vi "_Subsystem_Name Build Trace String.vi"(10 "Current Command":T1, 11 "Initial Trace String":string) -> (3 "Trace String":string)   [LabVIEW 2023]
doc: "This VI is called to construct a trace string from the command arguments."
uses:
  _Subsystem_Name Operations.ctl
  _Subsystem_Name Setpoints.ctl
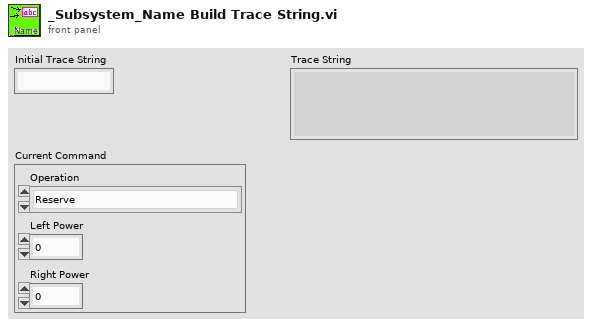
[diagram p1: front panel]
types:
  T1 = typedef "_Subsystem_Name Setpoints.ctl" = cluster{"Operation":T2, "Left Power":dbl, "Right Power":dbl}
  T2 = typedef "_Subsystem_Name Operations.ctl" = enum16{"Reserve", "Read Current", "Immediate"}
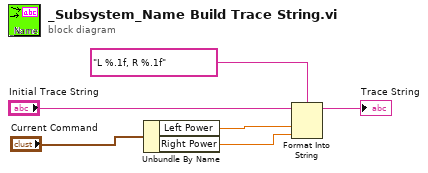
[diagram p0: block diagram]
diagram:
  n1 = Unbundle By Name("Current Command") -> ("Left Power"=w1:dbl, "Right Power"=w6:dbl)
  n2 = Format Into String(format string="L %.1f, R %.1f", initial string="Initial Trace String", w1, w6) -> (resulting string=→"Trace String":string)  [unwired: 1 in, 1 out]
